vi "Lab06_task3_OverSampling.vi"() -> ()   [LabVIEW 2022 SP3]
uses:
  <vilib>/DAQmx/read.llb/DAQmx Read (Analog 2D I16 NChan NSamp).vi
  <vilib>/Analysis/2dsp.llb/Decimate (single shot, DBL).vi
  <vilib>/DAQmx/create/channels.llb/DAQmx Create Channel (AI-Voltage-Basic).vi
  <vilib>/DAQmx/configure/timing.llb/DAQmx Timing (Sample Clock).vi
  <vilib>/DAQmx/miscellaneous.llb/DAQmx Fill In Error Info.vi
  <vilib>/express/express analysis/Spectral/Block/exnSpectralBlock spectral measurements RMS poly.vi
  <vilib>/express/express analysis/Spectral/Block/exnSpectralBlock spectral measurements RMS WFM.vi
  <vilib>/express/express analysis/Spectral/XNode/ExpressSpectralMeasurementsBlockNode.xnode
  <vilib>/measure/NI_MABase.lvlib
  <vilib>/Analysis/NI_AALPro.lvlib
panel:
  out "Waveform Graph":dbl[](graph)
  out "Decimated Array":dbl[](array[numeric])
  in  "decimating factor":i32=1
  in  "nr of samples":i32=5000
  in  "input channel":tag="Dev1/ai0"
  in  "rate":dbl=3000.0 format="%#_13g"
  in  "stop write loop":bool
  in  "dither  amplitude":dbl format="%.2p"
  in  "output device name":tag="Dev1"
  in  "stop read loop":bool
  out "full 16 bit signal":i16[](graph)
  out "Low resolution ADC signal":i16[](graph)
  out "FFT of low resolution ADC":cluster{"f0":dbl, "df":dbl, "magnitude":dbl[]}(graph)={"f0"=0.0, "df"=0.6000000000000001, "magnitude"=[]}
  in  "ADC number of bits":i32=1
  out "full 16 bit signal\n(binary view)":i16[](array[numeric]) format="%016b"
  out "Low resolution ADC signal\n(binary view)":i16[](array[numeric]) format="%016b"
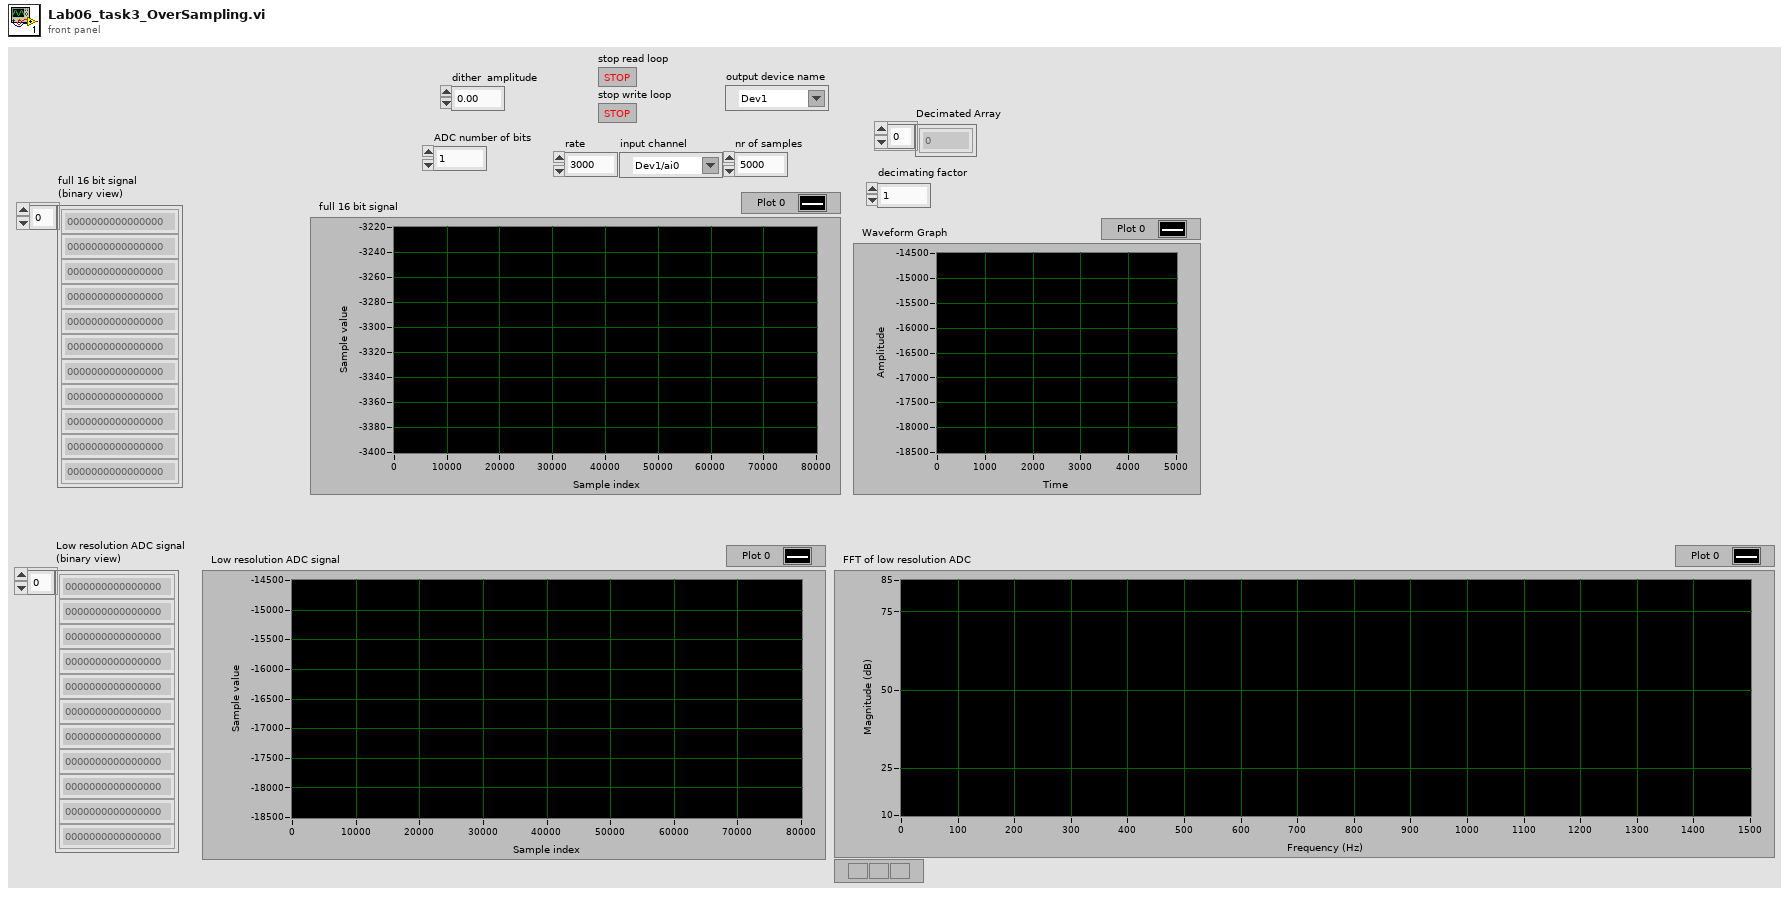
[diagram p1: front panel]
types:
  T1 = cluster{"averaging mode":u16, "weighting mode":u16, "number of averages":u32}
  T2 = cluster{"dB On (F)":bool, "unwrap phase (F)":bool, "convert to degree (F)":bool}
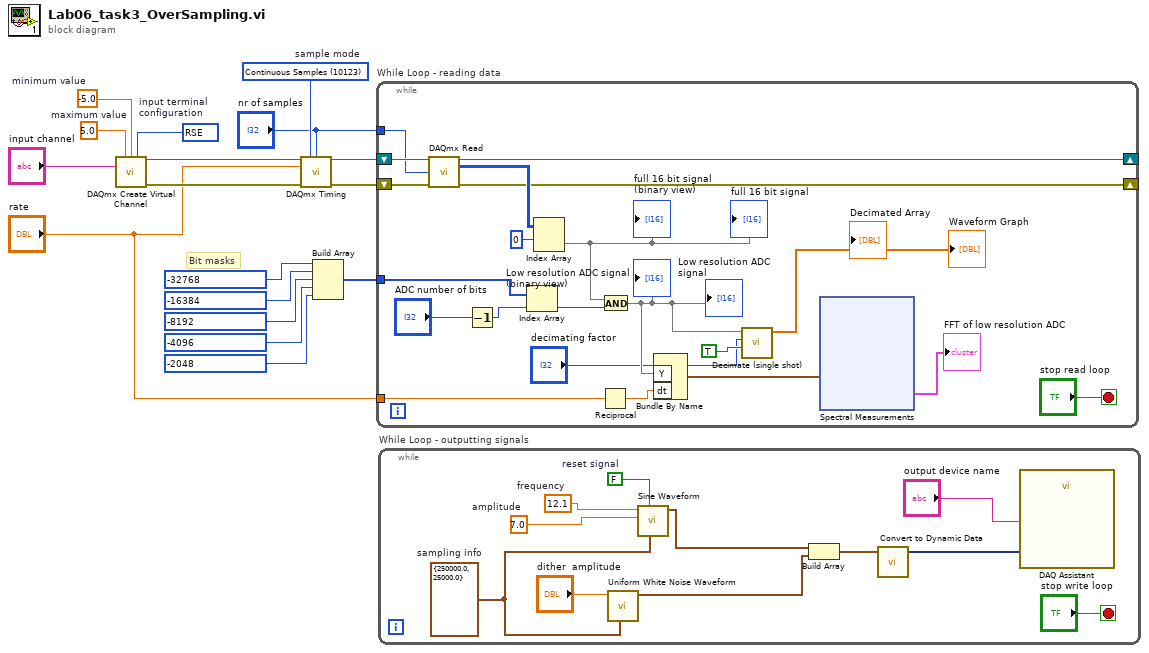
[diagram p0: block diagram]
diagram:
  w9 = 10123 items=["Finite Samples"=10178, "Continuous Samples"=10123, "Hardware Timed Single Point"=12522]  # sample mode
  w14 = 10083 items=["Default"=-1, "RSE"=10083, "NRSE"=10078, "Differential"=10106, "Pseudodifferential"=12529]  # input terminal  configuration
  w15 = 5.0  # maximum value
  w16 = -5.0  # minimum value
  # "Bit masks"
  n1 = call-poly <vilib>:"DAQmx Create Virtual Channel.vi"("maximum value"=w15, "minimum value"=w16, "input terminal configuration"=w14, "physical channels"="input channel") -> ("task out"=w13:refnum<k21>, "error out"=w11:errorcluster)  [unwired: 10 in]
  n2 = call-poly <vilib>:"DAQmx Timing.vi"("task/channels in"=w13, "sample mode"=w9, "samples per channel"="nr of samples", "rate"="rate", "error in"=w11) -> ("task out"=w12:refnum<k21>, "error out"=w10:errorcluster)  [unwired: 9 in]
  n3 = Build Array "Build Array"(i16 -32768 ("y"), i16 -16384 ("y"), i16 -8192 ("y"), i16 -4096 ("y"), i16 -2048 ("y")) -> (w2:i16[])
  n4 = while "While Loop - reading data" {
    shift-right: [w34] -> _
    shift-left: w10 -> [w37]
    shift-right: [w36] -> _
    shift-left: w12 -> [w38]
    tunnel: "rate" -> [w28]
    tunnel: w2 -> [w26]
    tunnel: "nr of samples" -> [w22]
    stop <- "stop read loop" stop-if-true
    n5 = call-poly <vilib>:"DAQmx Read.vi"("task/channels in"=w38, "number of samples per channel"=w22, "error in"=w37) -> ("task out"=w36:refnum<k21>, "data"=w35:i16[][], "error out"=w34:errorcluster)  [unwired: 10 in]
    n6 = Decrement(x="ADC number of bits") -> (x-1=w23:i32)
    n7 = Index Array "Index Array"(array=w26, index=w23) -> (element=w25:i16)
    n8 = Index Array "Index Array"(array=w35, index (row)=0) -> (element=w31:i16[])  [unwired: 1 in]
    "full 16 bit signal" <- w31
    "full 16 bit signal\n(binary view)" <- w31
    n9 = Reciprocal(x=w28) -> (1/x=w29:dbl)
    n10 = And(x=w31, y=w25) -> (x .and. y?=w21:i16[])
    "Low resolution ADC signal" <- w21
    "Low resolution ADC signal\n(binary view)" <- w21
    n11 = Bundle By Name("Y"=w21, "dt"=w29) -> (w27:waveform(i16))  [unwired: 1 in]
    n12 = call-poly <vilib>:"Decimate (single shot).vi"("averaging"=TRUE, "decimating factor"="decimating factor", "X"=w21) -> ("Decimated Array"=→"Decimated Array" →"Waveform Graph":dbl[])  [unwired: 7 in, 1 out]
    n13 = xnode "Spectral Measurements"("Signals"=w27) -> ("FFT - (RMS)"=→"FFT of low resolution ADC":cluster{"f0":dbl, "df":dbl, "magnitude":dbl[]})  [unwired: 1 in, 2 out]
  }
  n14 = while "While Loop - outputting signals" {
    stop <- "stop write loop" stop-if-true
    w57 = FALSE  # reset signal
    w53 = cluster{"Fs":dbl, "#s":dbl} {"Fs"=250000.0, "#s"=25000.0}  # sampling info
    w58 = 7.0  # amplitude
    w59 = 12.1  # frequency
    n15 = call <vilib>:"Uniform White Noise Waveform.vi"("sampling info"=w53, "amplitude"="dither  amplitude") -> ("signal out"=w54:waveform(dbl))  [unwired: 8 in, 1 out]
    n16 = call <vilib>:"Sine Waveform.vi"("sampling info"=w53, "reset signal"=w57, "amplitude"=w58, "frequency"=w59) -> ("signal out"=w56:waveform(dbl))  [unwired: 6 in, 1 out]
    n17 = Build Array "Build Array"(w56, w54) -> (w52:waveform(dbl)[])
    n18 = call "Convert to Dynamic Data"("Array of Waveforms"=w52) -> ("Dynamic Data Type"=w51:dynamicdata)  [unwired: 3 in]
    n19 = call "DAQ Assistant"("data"=w51, "device name"="output device name") -> ()  [unwired: 15 in, 3 out]
  }
